vi "Gear_Rail.vi"(0 "MotorControlDevRef":T4={"DeviceStatus"={"status"=FALSE, "code"=0, "source"=""}, "Type"=enum."PWM", "PWM"={"PWM Channel"=enum."Invalid", "DeadBand"={"Name"="", "maxPositivePwm"=0, "minPositivePwm"=0, "centerPwm"=0, "maxNegativePwm"=0, "minNegativePwm"=0, "angularRange"=0}}, "CAN"={"Device Number"=0, "SetOutput VI Ref"=variant(refnum<vi> refnum), "GetOutput VI Ref"=variant(refnum<vi> refnum), "Enable VI Ref"=variant(refnum<vi> refnum), "Disable VI Ref"=variant(refnum<vi> refnum), "Data"=variant}, "Invert"=FALSE}, 1 "dt_In_PID":dbl=-1.0 format="%.3f", 2 "Potentiometer_Input":dbl, 3 "Potentiometer_WantedPos":dbl(slide) scale=0.0..30.0, 4 "Motor_Input":dbl, 5 "Rail Parameters":T1={"Scale Positions"={"Forward_StartScale"=0.0, "Reverse_StartScale"=0.0, "Forward_Limit"=0.0, "Reverse_Limit"=0.0}, "Motor_Limit"=0.6, "Invert?"=FALSE, "PID gains"={"proportional gain (Kc)"=1.0, "integral time (Ti, min)"=0.01, "derivative time (Td, min)"=0.0}, "Timeout (ms)"=2000, "CatchPosition"=6.5} {"PID gains"."derivative time (Td, min)" format="%.3f"; "PID gains"."integral time (Ti, min)" format="%.3f"; "PID gains"."proportional gain (Kc)" format="%.3f"}) -> (20 "dt_Out_PID":dbl format="%.3f")   [LabVIEW 2016]
uses:
  <vilib>/Rock Robotics/WPI/MotorControl/WPI_MotorControlDeviceRef.ctl
  <vilib>/Rock Robotics/WPI/MotorControl/WPI_MotorControlType.ctl
  <vilib>/Rock Robotics/SystemInterfaces/DIO/FPGA_DIOPWMChannel.ctl
  <vilib>/Rock Robotics/WPI/PWM/WPI_PWMDeadband.ctl
  TypeDefs/RailParameters_Type.ctl
  ArgosLib/Miscellaneous/TypeDefs/MotorLimitPositions_Type.ctl
  ArgosLib/Signal Processing/TypeDefs/EdgeDetector_Type.ctl
  <vilib>/addons/control/pid/pid.llb/PID (DBL).vi
  Global_Var-RefNum/Global_Var_Other.vi
  <vilib>/addons/control/pid/NI_PID_pid.lvlib
  ArgosLib/ArgosLib.lvlib
panel:
  out "Waveform Chart":T3(graph)
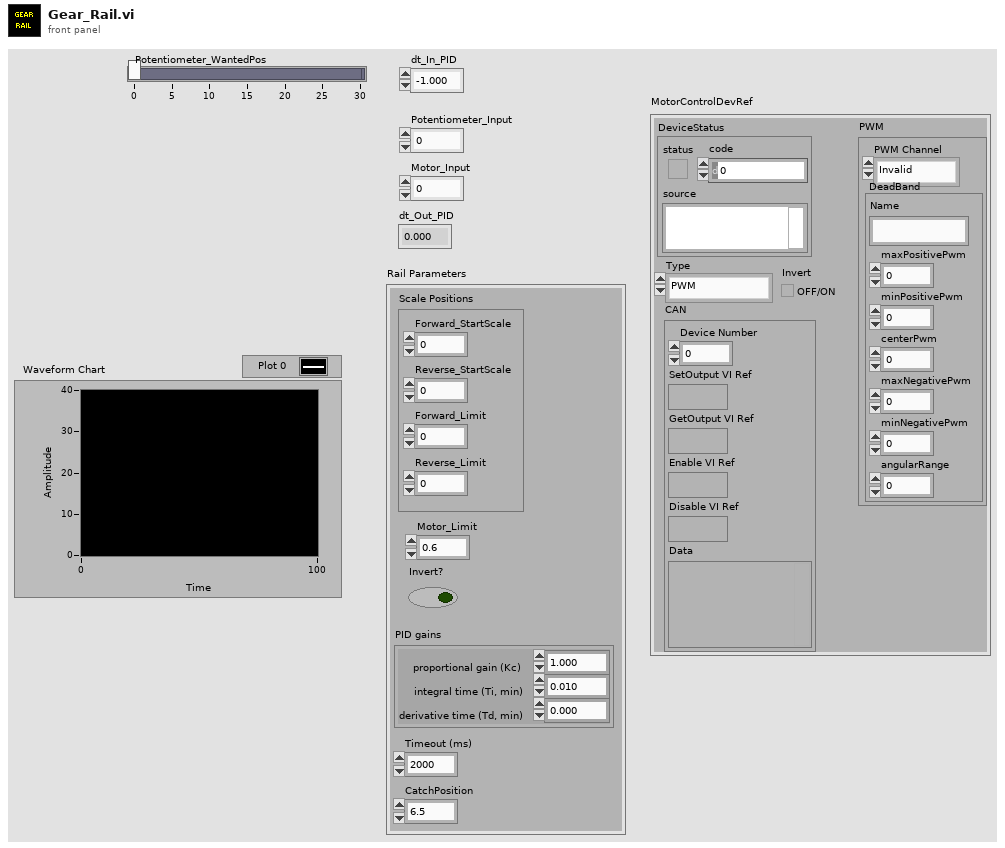
[diagram p1: front panel]
types:
  T1 = typedef "RailParameters_Type.ctl" = cluster{"Scale Positions":T2, "Motor_Limit":dbl, "Invert?":bool, "PID gains":cluster{"proportional gain (Kc)":dbl, "integral time (Ti, min)":dbl, "derivative time (Td, min)":dbl}, "Timeout (ms)":u32, "CatchPosition":dbl}
  T2 = typedef "MotorLimitPositions_Type.ctl" = cluster{"Forward_StartScale":dbl, "Reverse_StartScale":dbl, "Forward_Limit":dbl, "Reverse_Limit":dbl}
  T3 = cluster{"Potentiometer_Input":dbl, "Potentiometer_WantedPos":dbl}
  T4 = typedef "WPI_MotorControlDeviceRef.ctl" = cluster{"DeviceStatus":errorcluster, "Type":T5, "PWM":cluster{"PWM Channel":T6, "DeadBand":T7}, "CAN":cluster{"Device Number":u8, "SetOutput VI Ref":variant, "GetOutput VI Ref":variant, "Enable VI Ref":variant, "Disable VI Ref":variant, "Data":variant}, "Invert":bool}
  T5 = typedef "WPI_MotorControlType.ctl" = enum16{"PWM", "CAN"}
  T6 = typedef "FPGA_DIOPWMChannel.ctl" = enum8{"PWM 0", "PWM 1", "PWM 2", "PWM 3", "PWM 4", "PWM 5", "PWM 6", "PWM 7", "PWM 8", "PWM 9", "PWM MXP 0", "PWM MXP 1", "PWM MXP 2", "PWM MXP 3", "PWM MXP 4", "PWM MXP 5", "PWM MXP 6", "PWM MXP 7", "PWM MXP 8", "PWM MXP 9", "Invalid"}
  T7 = typedef "WPI_PWMDeadband.ctl" = cluster{"Name":string, "maxPositivePwm":i32, "minPositivePwm":i32, "centerPwm":i32, "maxNegativePwm":i32, "minNegativePwm":i32, "angularRange":u16}
  T8 = typedef "EdgeDetector_Type.ctl" = enum16{"RisingEdge", "FallingEdge", "Both"}
  T9 = cluster{"proportional gain (Kc)":dbl, "integral time (Ti, min)":dbl, "derivative time (Td, min)":dbl}
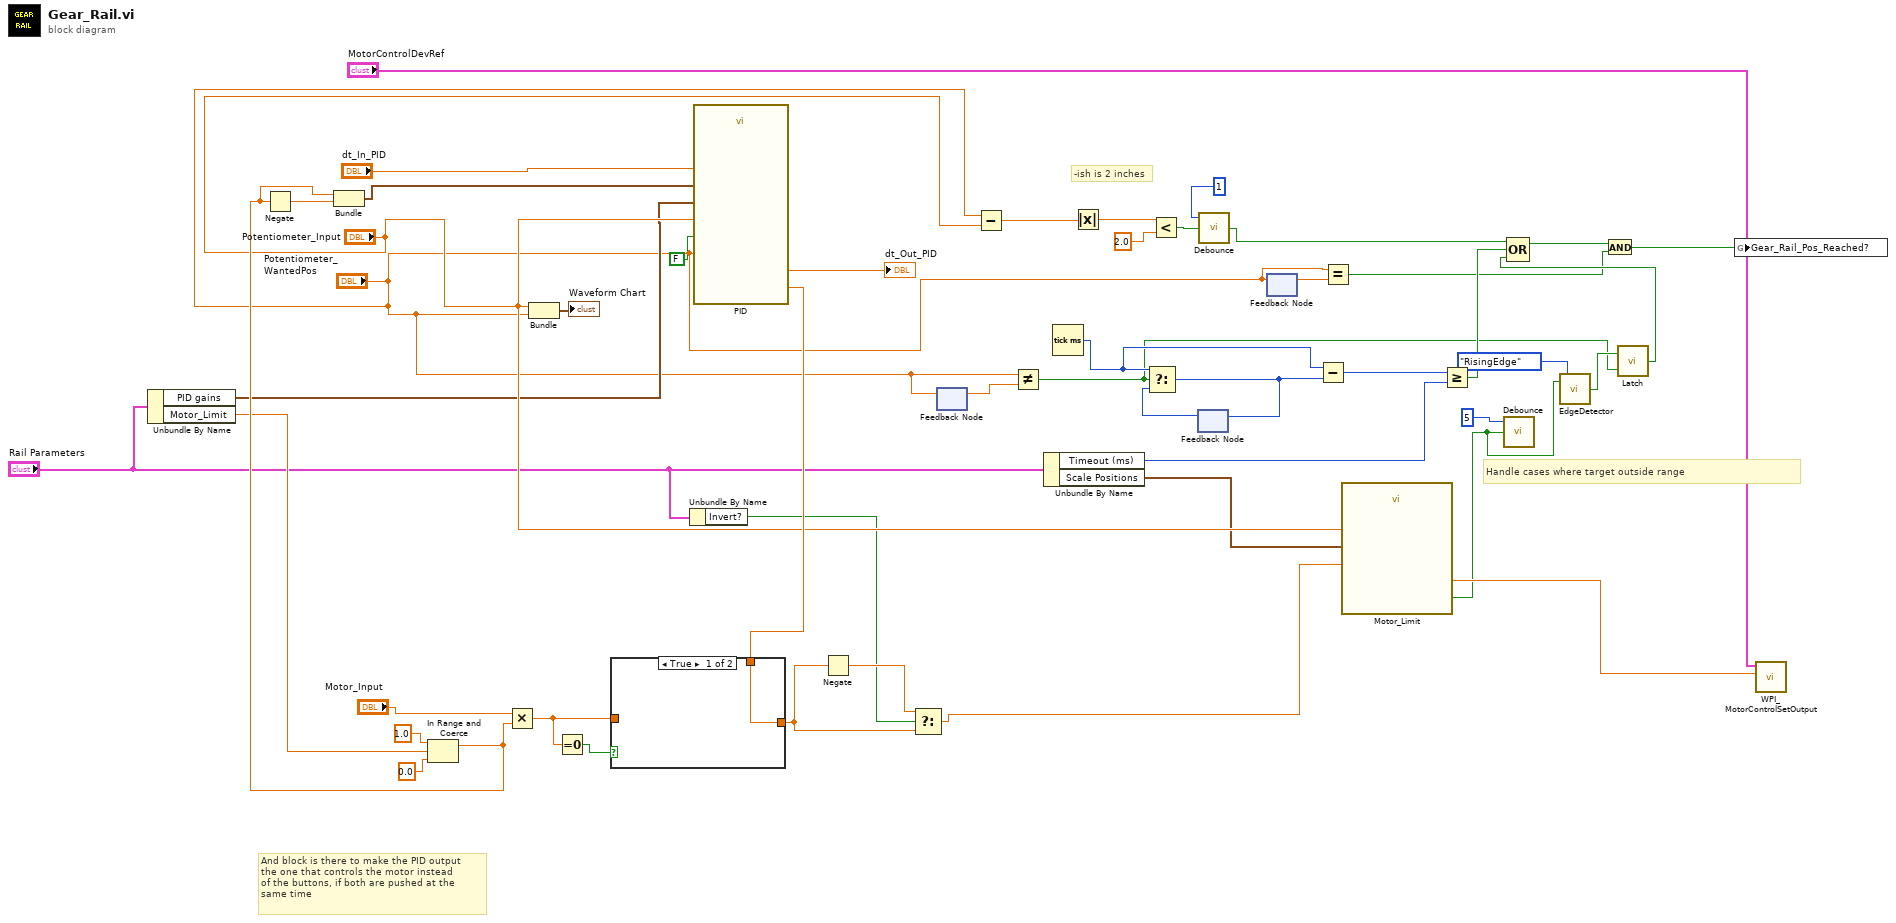
[diagram p0: block diagram]
diagram:
  # "Handle cases where target outside range"
  # "-ish is 2 inches"
  # "And block is there to make the PID output \nthe one that controls the motor instead\nof the buttons, if both are pushed at the \nsame time"
  n1 = Unbundle By Name("Rail Parameters") -> ("PID gains"=w16:T9, "Motor_Limit"=w15:dbl)
  n2 = In Range and Coerce(upper limit=1.0, x=w15, lower limit=0.0) -> (coerced(x)=w27:dbl)  [unwired: 1 out]
  n3 = Negate(x=w27) -> (-x=w31:dbl)
  n4 = Bundle("upper limit"=w27, w31) -> (w30:cluster{"upper limit":dbl, dbl})  [unwired: 1 in]
  n5 = Multiply(x="Motor_Input", y=w27) -> (x*y=w33:dbl)
  n6 = Bundle("Potentiometer_Input"="Potentiometer_Input", "Potentiometer_WantedPos"="Potentiometer_WantedPos") -> (→"Waveform Chart":T3)  [unwired: 1 in]
  n7 = Equal To 0?(x=w33) -> (x = 0?=w32:bool)
  n8 = Unbundle By Name("Rail Parameters") -> ("Invert?"=w14:bool)
  n9 = call-poly <vilib>:"PID.vi"("reinitialize? (F)"=FALSE, "output range"=w30, "dt (s)"="dt_In_PID", "PID gains"=w16, "process variable"="Potentiometer_Input", "setpoint"="Potentiometer_WantedPos") -> ("dt out (s)"=→"dt_Out_PID":dbl, "output"=w39:dbl)  [unwired: 4 in]
  n10 = case shown="True" w32 {
    tunnel: [w49 w50] -> w46
    tunnel: w39 -> [w49 _]
    tunnel: w33 -> [_ w50]
    frame True {
    }
    frame False {
    }
  }
  n11 = Negate(x=w46) -> (-x=w48:dbl)
  n12 = Select(t=w48, s=w14, f=w46) -> (s? t:f=w35:dbl)
  n13 = feedback-in #1("Potentiometer_WantedPos") -> ()
  n14 = feedback #1() -> (w24:dbl)  [unwired: 1 in]
  n15 = Subtract(x="Potentiometer_WantedPos", y="Potentiometer_Input") -> (x-y=w40:dbl)
  n16 = Not Equal?(x="Potentiometer_WantedPos", y=w24) -> (x != y?=w6:bool)
  n17 = Unbundle By Name("Rail Parameters") -> ("Timeout (ms)"=w12:u32, "Scale Positions"=w11:T2)
  n18 = Tick Count (ms)() -> (millisecond timer value=w21:u32)
  n19 = Absolute Value(x=w40) -> (abs(x)=w41:dbl)
  n20 = Less?(x=w41, y=2.0) -> (x < y?=w38:bool)
  n21 = feedback #2() -> (w23:u32)  [unwired: 1 in]
  n22 = Select(t=w21, s=w6, f=w23) -> (s? t:f=w22:u32)
  n23 = feedback-in #2(w22) -> ()
  n24 = call "Debounce.vi"("Input"=w38, "Num samples"=1) -> ("Output"=w17:bool)  [unwired: 1 in]
  n25 = feedback-in #3("Potentiometer_WantedPos") -> ()
  n26 = feedback #3() -> (w4:dbl)  [unwired: 1 in]
  n27 = Subtract(x=w21, y=w22) -> (x-y=w20:u32)
  n28 = Equal?(x="Potentiometer_WantedPos", y=w4) -> (x = y?=w1:bool)
  n29 = call "Motor_Limit.vi"("Current_Pos"="Potentiometer_Input", "Motor_Speed"=w35, "Scale Positions"=w11) -> ("New_Motor_Speed"=w36:dbl, "At Limit"=w9:bool)  [unwired: 15 in]
  n30 = Greater Or Equal?(x=w20, y=w12) -> (x >= y?=w18:bool)
  n31 = call "Debounce.vi"("Input"=w9, "Num samples"=5) -> ()  [unwired: 1 in, 1 out]
  n32 = call "EdgeDetector.vi"("DetectorType"=EdgeDetector_Type."RisingEdge", "Input"=w9) -> ("Edge"=w7:bool)
  n33 = call "Latch.vi"("Reset"=w6, "Input"=w7) -> ("LatchOut"=w5:bool)
  n34 = Compound Arithmetic op=OR(w17, w18, w5) -> (w19:bool)
  n35 = And(x=w19, y=w1) -> (x .and. y?=w2:bool)
  n36 = global write "Global_Var_Other.vi" "Gear_Rail_Pos_Reached?"(w2) -> ()
  n37 = call <vilib>:"WPI_MotorControlSetOutput.vi"("Output"=w36, "MotorControlDevRef"="MotorControlDevRef") -> ()  [unwired: 7 in, 3 out]
